vi "Read Message.vi"(8 "error in (no error)":errorcluster, 11 "CLI in":refnum<class "CLI.lvclass">) -> (0 "error out":errorcluster, 1 "Message Contents":string, 2 "Message Type":string, 3 "CLI out":refnum<class "CLI.lvclass">)   [LabVIEW 2015, in "CLI.lvclass"]
uses:
  CLI.lvclass
  CLI.lvclass/CLI.ctl
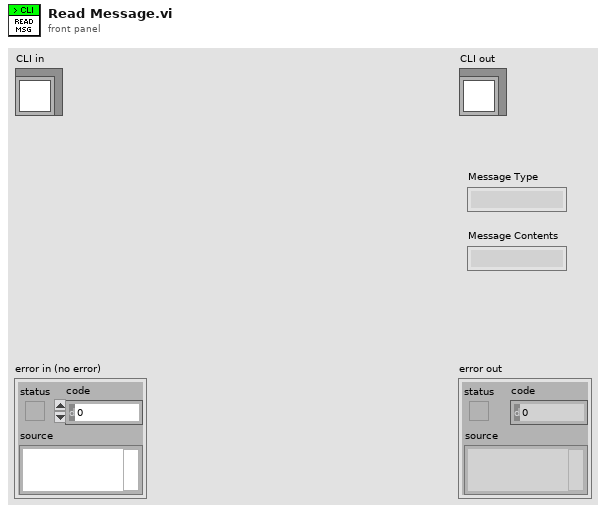
[diagram p1: front panel]
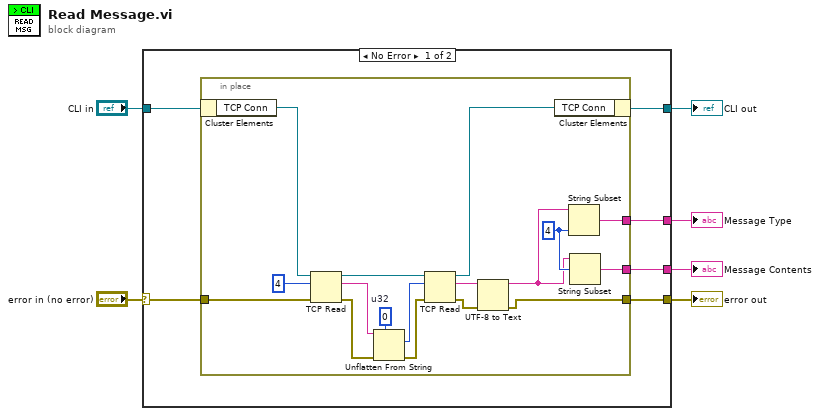
[diagram p0: block diagram]
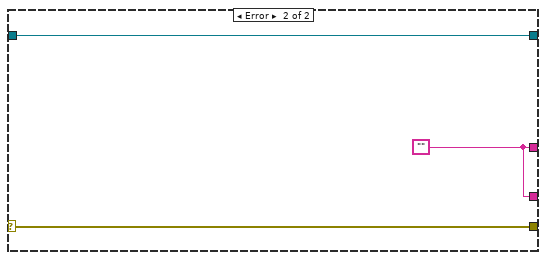
[diagram p2: hidden frame]
diagram:
  n1 = case shown="No Error" "error in (no error)" {
    selector: "error in (no error)" -> [w12 w32]
    tunnel: [w10 w32] -> w5
    tunnel: [w9 w31] -> w3
    tunnel: "CLI in" -> [w11 w31]
    tunnel: [w8 w30] -> w2
    tunnel: [w7 w30] -> w1
    frame No Error {
      n2 = in-place {
        in-place-border: w12 -> [w28]
        in-place-border: [w17] -> w10
        in-place-border: [w18] -> w8
        in-place-border: [w16] -> w7
        w19 = 4 ("length (rest)")
        w21 = 0  # u32
        n3 = in-place-cluster #1(w11) -> ("TCP Conn"=w29:refnum<k5>)
        n4 = TCP Read(connection ID=w29, bytes to read=4, error in (no error)=w28) -> (connection ID out=w26:refnum<k5>, data out=w22:string, error out=w27:errorcluster)  [unwired: 2 in]
        n5 = Unflatten From String(type=w21, binary string=w22, error in (no error)=w27) -> (value=w20:i32, error out=w23:errorcluster)  [unwired: 2 in, 1 out]
        n6 = TCP Read(connection ID=w26, bytes to read=w20, error in (no error)=w23) -> (connection ID out=w25:refnum<k5>, data out=w15:string, error out=w14:errorcluster)  [unwired: 2 in]
        n7 = UTF-8 to Text(8:w14, 11:w15) -> (0:w17:errorcluster, 3:w13:string)  [unwired: 1 in]
        n8 = in-place-cluster #1("TCP Conn"=w25) -> (w9:refnum<class "CLI.lvclass">)
        n9 = String Subset(string=w13, length (rest)=w19) -> (substring=w18:string)  [unwired: 1 in]
        n10 = String Subset(string=w13, offset (0)=w19) -> (substring=w16:string)  [unwired: 1 in]
      }
    }
    frame Error {
      w30 = ""
    }
  }
  "error out" <- w5
  "CLI out" <- w3
  "Message Type" <- w2
  "Message Contents" <- w1
